vi "ErrBool A.vi"(0 "flag":bool, 11 "error in":errorcluster) -> (4 "no error?":bool, 6 "error or flag?":bool, 8 "which frame":string)   [LabVIEW 2026]
doc: "Probe: an error cluster wired straight into Not, Or and a Case selector."
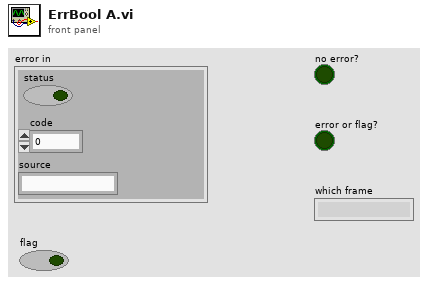
[diagram p1: front panel]
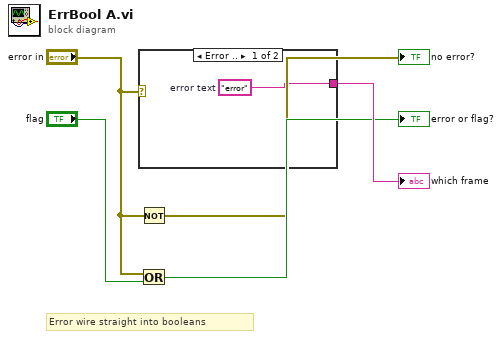
[diagram p0: block diagram]
diagram:
  # "Error wire straight into booleans"
  n1 = case shown="Error .." "error in" {
    tunnel: [w6 w7] -> w5
    frame Error {
      w6 = "error"  # error text
    }
    frame No Error {
      w7 = "ok"  # ok text
    }
  }
  "which frame" <- w5
  n2 = Not(x="error in") -> (.not. x?=→"no error?":errorcluster)
  n3 = Or(x="error in", y="flag") -> (x .or. y?=→"error or flag?":bool)
